vi "Add Argument Integer.vi"(8 "error in (no error)":errorcluster, 9 "value":i32, 10 "key":string, 11 "reference":refnum<k24>) -> (0 "error out":errorcluster, 3 "reference out":refnum<k24>)   [LabVIEW 2026, in "ToastNotification.lvlib" / "Toast Native.lvlib"]
doc: "Native AddArgument integer overload. Add an Int64 activation argument to a borrowed ToastContentBuilder. reference out aliases the input; no builder handle is created or closed. Arguments are distinct from displayed text and submitted UserInput."
uses:
  Toast Native.lvlib
  C:/Users/loicw/Documents/LabVIEW/ToastNotifications/Sources/bins/Microsoft.Toolkit.Uwp.Notifications.dll
  bins/Microsoft.Toolkit.Uwp.Notifications.dll
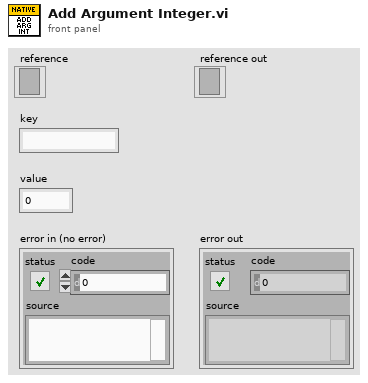
[diagram p1: front panel]
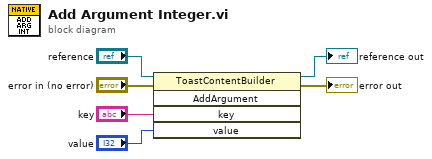
[diagram p0: block diagram]
diagram:
  n1 = invoke class="ToastContentBuilder" method="AddArgument"(reference="reference", error in="error in (no error)", "key"="key", "value"="value") -> (reference out=→"reference out":refnum<k24>, error out=→"error out":errorcluster)  [unwired: 1 in, 3 out]
